vi "Bridge_Validate_Command.vi"(8 "error in (no error)":errorcluster={"status"=FALSE, "code"=0, "source"="\"\""}, 10 "active plan":string, 11 "CommandRequest":string) -> (0 "error out":errorcluster={"status"=FALSE, "code"=0, "source"="\"\""}, 2 "status ok":bool, 3 "Authorized/rejected reason":string)   [LabVIEW 2026]
doc: "INTENT: Validate command setpoint against rig limits and clamp if within authorized envelope."
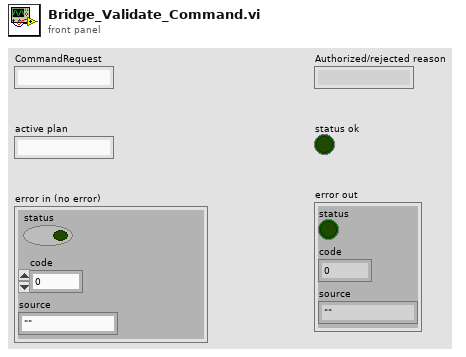
[diagram p1: front panel]
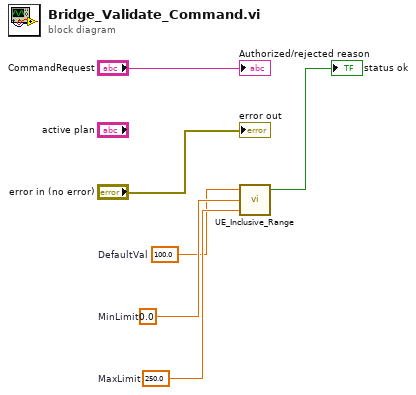
[diagram p0: block diagram]
diagram:
  w5 = 250.0  # MaxLimit
  w4 = 0.0  # MinLimit
  w3 = 100.0  # DefaultVal
  n1 = call "UE_Inclusive_Range.vi"("maximum"=w5, "minimum"=w4, "value"=w3) -> ("in_range"=→"status ok":bool)  [unwired: 2 in]
  "Authorized/rejected reason" <- "CommandRequest"
  "error out" <- "error in (no error)"
